vi "Build Step Table.vi"(10 "Step Results":T1[](array[typedef]), 11 "Sequence File":T2) -> (3 "Step Table":string[][](array[string]))   [LabVIEW 2026]
doc: "Builds the step table for display: one row per step of the Sequence File with the columns Step, Name, Command, Monitored IO, Target, Tol, Dwell ms, Timeout ms, Result, Measured, Duration ms, Reason. Target is the setpoint of the step's monitored signal. Result, Measured, Duration ms and Reason come from the Step Result with the same index; a step without a result shows empty result text and zeros. Pure function, no error terminals, AF-free."
uses:
  Typedefs/Sequence File.ctl
  Typedefs/Step Config.ctl
  Typedefs/Step Result.ctl
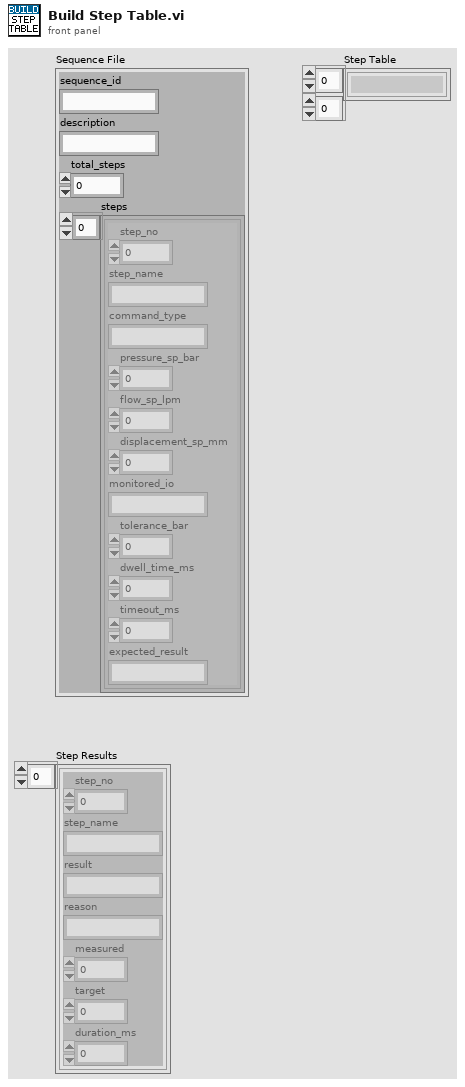
[diagram p1: front panel]
types:
  T1 = typedef "Step Result.ctl" = cluster{"step_no":i32, "step_name":string, "result":string, "reason":string, "measured":dbl, "target":dbl, "duration_ms":dbl}
  T2 = typedef "Sequence File.ctl" = cluster{"sequence_id":string, "description":string, "total_steps":i32, "steps":T3[]}
  T3 = typedef "Step Config.ctl" = cluster{"step_no":i32, "step_name":string, "command_type":string, "pressure_sp_bar":dbl, "flow_sp_lpm":dbl, "displacement_sp_mm":dbl, "monitored_io":string, "tolerance_bar":dbl, "dwell_time_ms":i32, "timeout_ms":i32, "expected_result":string}
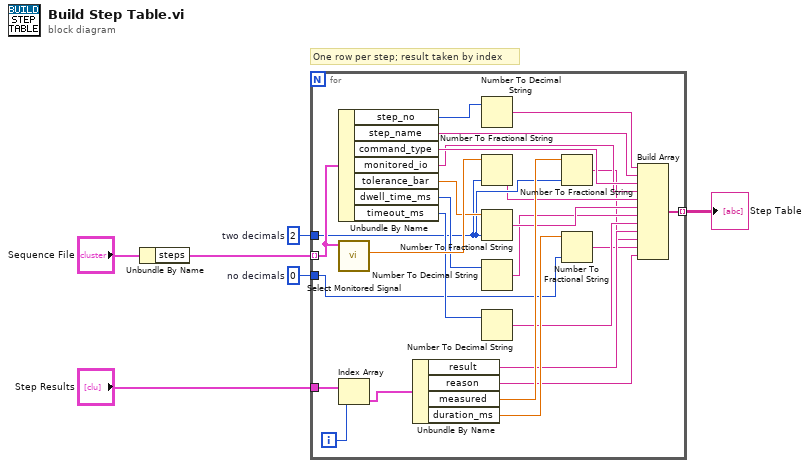
[diagram p0: block diagram]
diagram:
  w2 = 0  # no decimals
  w3 = 2  # two decimals
  # "One row per step; result taken by index"
  n1 = Unbundle By Name("Sequence File") -> ("steps"=w5:T3[])
  n2 = for {
    tunnel: w5 -> [w32] mode=indexing
    tunnel: "Step Results" -> [w31]
    tunnel: w3 -> [w23]
    tunnel: w2 -> [w21]
    tunnel: [w8] -> w1 mode=indexing
    i -> [w7]
    n3 = Unbundle By Name(w32) -> ("step_no"=w29:i32, "step_name"=w19:string, "command_type"=w18:string, "monitored_io"=w17:string, "tolerance_bar"=w27:dbl, "dwell_time_ms"=w26:i32, "timeout_ms"=w25:i32)
    n4 = call "Select Monitored Signal.vi"("Step Config"=w32) -> ("target"=w28:dbl)  [unwired: 8 in, 2 out]
    n5 = Index Array(array=w31, index=w7) -> (element=w30:T1)
    n6 = Unbundle By Name(w30) -> ("result"=w12:string, "reason"=w9:string, "measured"=w24:dbl, "duration_ms"=w22:dbl)
    n7 = Number To Decimal String(number=w29) -> (decimal integer string=w20:string)  [unwired: 1 in]
    n8 = Number To Fractional String(number=w28, precision (6)=w23) -> (F-format string=w16:string)  [unwired: 2 in]
    n9 = Number To Fractional String(number=w27, precision (6)=w23) -> (F-format string=w15:string)  [unwired: 2 in]
    n10 = Number To Decimal String(number=w26) -> (decimal integer string=w14:string)  [unwired: 1 in]
    n11 = Number To Decimal String(number=w25) -> (decimal integer string=w13:string)  [unwired: 1 in]
    n12 = Number To Fractional String(number=w24, precision (6)=w23) -> (F-format string=w11:string)  [unwired: 2 in]
    n13 = Number To Fractional String(number=w22, precision (6)=w21) -> (F-format string=w10:string)  [unwired: 2 in]
    n14 = Build Array(w20, w19, w18, w17, w16, w15, w14, w13, w12, w11, w10, w9) -> (w8:string[])
  }
  "Step Table" <- w1
